vi "Build CE Deployment.vi"(4 "Exclude file name patterns":string, 5 "preserve current version code (T)":bool=TRUE, 6 "Folders":string="Examples\nHelp\nProject\nTemplates\nvi.lib", 7 "Exclude undesired paths (T)":bool=TRUE, 8 "error in":errorcluster, 9 "LV Version":string(combo)="14.0", 10 "Target Dir":path, 11 "Source Dir":path) -> (0 "error out":errorcluster, 1 "Excluded Paths":path[](array[path]), 2 "dup Target Dir":path, 3 "dup Source Dir":path)   [LabVIEW 2021]
doc: "::: CalcExpress Toolkit :::\nCopyright (c) 2000-2026 Konstantin Shifershteyn. All rights reserved."
panel:
  # "CalcExpress Toolkit\nCopyright (c) 2000-2026 Konstantin Shifershteyn"
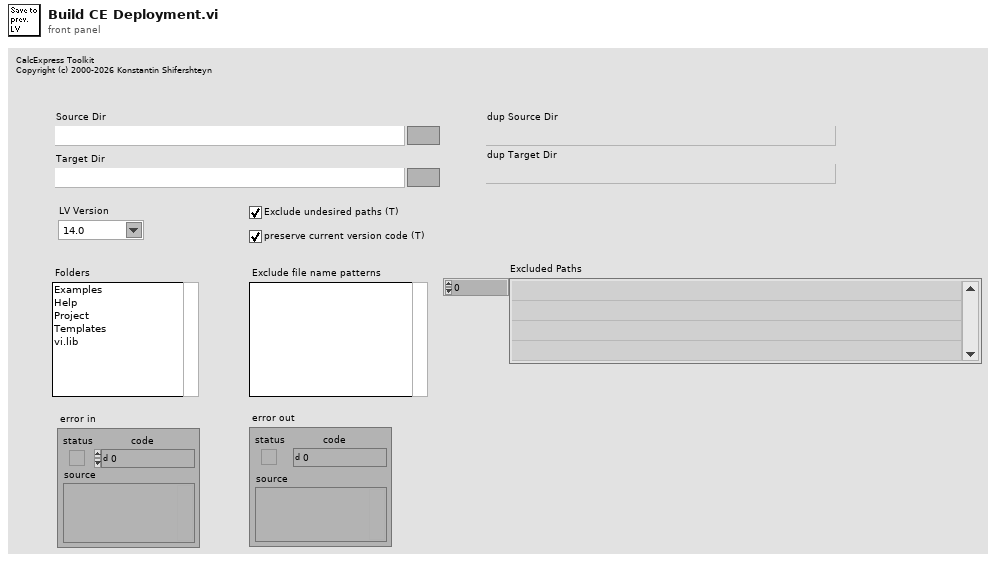
[diagram p1: front panel]
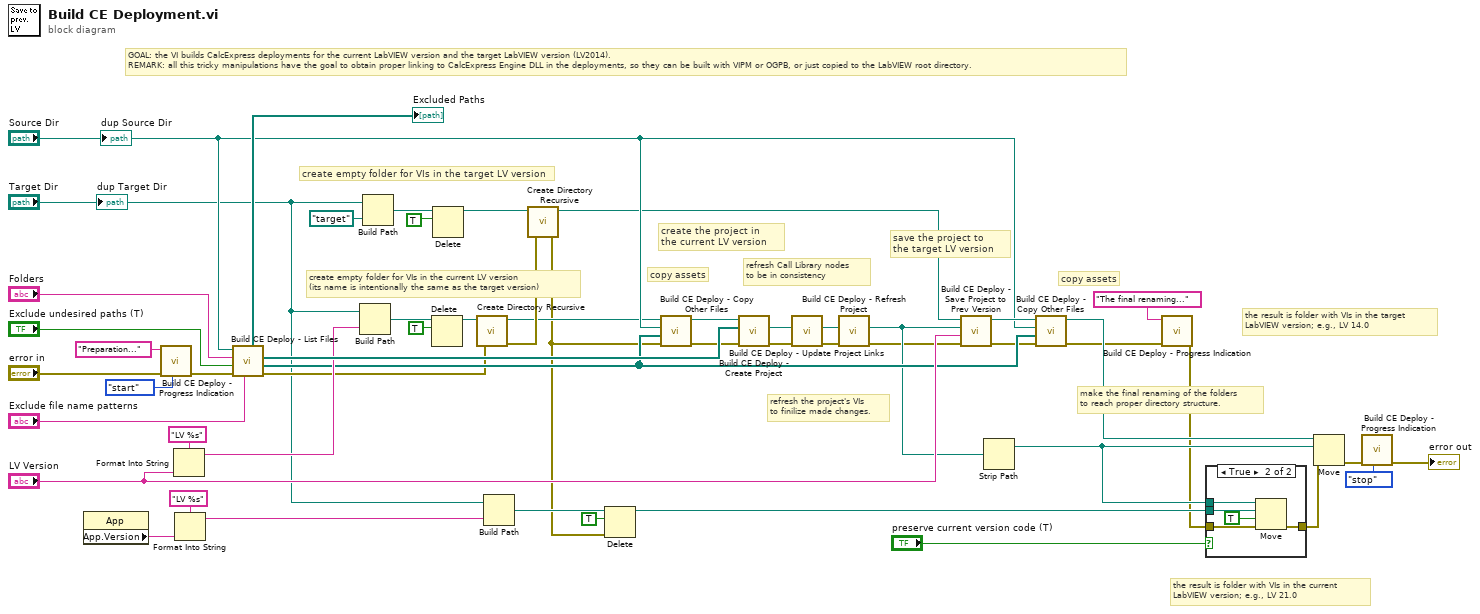
[diagram p0: block diagram]
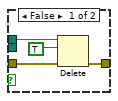
[diagram p2: hidden frame]
diagram:
  # "GOAL: the VI builds CalcExpress deployments for the current LabVIEW version and the target LabVIEW version (LV2014).\nREMARK: all this tricky manipulations have the goal to obtain proper linking to CalcExpress Engine DLL in the deployments, so they can be built with VIPM or OGPB, or just copied to the LabVIEW root directory."
  # "the result is folder with VIs in the target\nLabVIEW version; e.g., LV 14.0"
  # "the result is folder with VIs in the current\nLabVIEW version; e.g., LV 21.0"
  # "refresh the project's VIs\nto finilize made changes."
  # "refresh Call Library nodes\nto be in consistency"
  # "create the project in\nthe current LV version"
  # "copy assets"
  # "save the project to\nthe target LV version"
  # "copy assets"
  # "make the final renaming of the folders\nto reach proper directory structure."
  # "create empty folder for VIs in the current LV version\n(its name is intentionally the same as the target version)"
  # "create empty folder for VIs in the target LV version"
  n1 = property class="App"() -> ("App.Version"=w20:string)  [unwired: 2 in, 2 out]
  n2 = call "Build CE Deploy - Progress Indication.vi"("mode (run)"=enum16{"run", "start", "stop"}."start", "error in"="error in", "message 1"="Preparation...") -> ("error out"=w9:errorcluster)  [unwired: 8 in]
  n3 = Format Into String(format string="LV %s", "LV Version") -> (resulting string=w46:string)  [unwired: 2 in, 1 out]
  n4 = Format Into String(format string="LV %s", w20) -> (resulting string=w17:string)  [unwired: 2 in, 1 out]
  n5 = call "Build CE Deploy - List Files.vi"("Exclude file names"="Exclude file name patterns", "error in"=w9, "Exclude undesired paths (F)"="Exclude undesired paths (T)", "Folders"="Folders", "Source Dir"="Source Dir") -> ("error out"=w29:errorcluster, "Files to Copy"=w38:path[], "Project Files"=w53:path[], "Excluded Paths"=→"Excluded Paths":path[])  [unwired: 2 in, 1 out]
  n6 = Build Path(base path="Target Dir", name or relative path=w46) -> (appended path=w31:path)
  n7 = Build Path(base path="Target Dir", name or relative path=path "target") -> (appended path=w28:path)
  n8 = Delete(path (use dialog)=w31, entire hierarchy (F)=TRUE) -> (deleted path=w30:path)  [unwired: 3 in, 2 out]
  n9 = Delete(path (use dialog)=w28, entire hierarchy (F)=TRUE) -> (deleted path=w27:path)  [unwired: 3 in, 2 out]
  n10 = call <vilib>:"Create Directory Recursive.vi"("error in (no error)"=w29, "directory"=w30) -> ("error out"=w25:errorcluster, "directory copy"=w24:path)  [unwired: 3 in, 1 out]
  n11 = Build Path(base path="Target Dir", name or relative path=w17) -> (appended path=w16:path)
  n12 = call <vilib>:"Create Directory Recursive.vi"("error in (no error)"=w25, "directory"=w27) -> ("error out"=w15:errorcluster, "directory copy"=w37:path)  [unwired: 3 in, 1 out]
  n13 = Delete(path (use dialog)=w16, entire hierarchy (F)=TRUE, error in=w15) -> (deleted path=w14:path)  [unwired: 2 in, 2 out]
  n14 = call "Build CE Deploy - Copy Other Files.vi"("error in"=w15, "Files to Copy"=w38, "Source Dir"="Source Dir", "Target Dir"=w24) -> ("error out"=w48:errorcluster, "dup Target Dir"=w49:path)  [unwired: 6 in]
  n15 = call "Build CE Deploy - Create Project.vi"("error in"=w48, "Project Files"=w53, "Target Dir"=w49) -> ("error out"=w42:errorcluster, "Project File Path"=w41:path)  [unwired: 6 in, 1 out]
  n16 = call "Build CE Deploy - Update Project Links.vi"("error in"=w42, "Project file"=w41) -> ("error out"=w34:errorcluster, "dup Project file"=w35:path)  [unwired: 8 in]
  n17 = call "Build CE Deploy - Refresh Project.vi"("error in"=w34, "Project file"=w35) -> ("error out"=w26:errorcluster, "dup Project file"=w33:path)  [unwired: 8 in]
  n18 = call "Build CE Deploy - Save Project to Prev Version.vi"("error in"=w26, "LV Version"="LV Version", "Project file"=w33, "Target Dir"=w37) -> ("error out"=w36:errorcluster, "dup Target Dir"=w40:path)  [unwired: 6 in]
  n19 = Strip Path(path=w33) -> (stripped path=w12:path)  [unwired: 1 out]
  n20 = call "Build CE Deploy - Copy Other Files.vi"("error in"=w36, "Files to Copy"=w38, "Source Dir"="Source Dir", "Target Dir"=w40) -> ("error out"=w3:errorcluster, "dup Target Dir"=w32:path)  [unwired: 6 in]
  n21 = call "Build CE Deploy - Progress Indication.vi"("error in"=w3, "message 1"="The final renaming...") -> ("error out"=w2:errorcluster)  [unwired: 9 in]
  n22 = case shown="True" "preserve current version code (T)" {
    tunnel: w14 -> [_ w62]
    tunnel: w2 -> [w57 w60]
    tunnel: [w56 w59] -> w13
    tunnel: w12 -> [w55 w58]
    frame False {
      n23 = Delete(path (use dialog)=w55, entire hierarchy (F)=TRUE, error in=w57) -> (error out=w56:errorcluster)  [unwired: 2 in, 2 out]
    }
    frame True {
      n24 = Move(source path=w58, error in=w60, 9:TRUE, 10:w62) -> (error out=w59:errorcluster)  [unwired: 1 in, 2 out]
    }
  }
  n25 = Move(source path=w32, error in=w13, 10:w12) -> (error out=w7:errorcluster)  [unwired: 2 in, 2 out]
  n26 = call "Build CE Deploy - Progress Indication.vi"("mode (run)"=enum16{"run", "start", "stop"}."stop", "error in"=w7) -> ("error out"=→"error out":errorcluster)  [unwired: 9 in]
  "dup Target Dir" <- "Target Dir"
  "dup Source Dir" <- "Source Dir"
